vi "Update UI row elements.vi"(8 "result":string="Pass", 9 "measured value":string="Started", 11 "input cluster":T1={"User name"="", "user account"="", "UI"=[], "DI"=[], "Barcode"="", "MCListbox Ref_in"=refnum, "sequence step #"=0, "Result?"=FALSE, "Report Path"=path "", "Test Sequence"=enum."Ensure all the connections are OK", "skip Test  "=[FALSE, FALSE, FALSE, FALSE, FALSE, FALSE, FALSE, FALSE, FALSE, FALSE, FALSE, FALSE, FALSE, FALSE, FALSE, FALSE, FALSE, FALSE, FALSE, FALSE, FALSE, FALSE, FALSE, FALSE, FALSE, FALSE, FALSE, FALSE, FALSE, FALSE, FALSE, FALSE]} {"DI"."Upper limit" format="%#_7f"; "DI"."Lower limit" format="%#_7f"}) -> (1 "Test status item names":string[][](array[string]), 3 "output cluster":T1={"User name"="", "user account"="", "UI"=[], "DI"=[], "Barcode"="", "MCListbox Ref_in"=refnum, "sequence step #"=0, "Result?"=FALSE, "Report Path"=path "", "Test Sequence"=enum."Ensure all the connections are OK", "skip Test  "=[FALSE, FALSE, FALSE, FALSE, FALSE, FALSE, FALSE, FALSE, FALSE, FALSE, FALSE, FALSE, FALSE, FALSE, FALSE, FALSE, FALSE, FALSE, FALSE, FALSE, FALSE, FALSE, FALSE, FALSE, FALSE, FALSE, FALSE, FALSE, FALSE, FALSE, FALSE, FALSE]} {"DI"."Upper limit" format="%#_7f"; "DI"."Lower limit" format="%#_7f"})   [LabVIEW 2021]
uses:
  5.ACTIVITIES/1.LabVIEW_State_Machine_Template/LabVIEW_State_Machine_Template/LabVIEW_State_Machine_Template/Project_Template/Queue Test updator/Controls/initialise cluster.ctl
  5.ACTIVITIES/1.LabVIEW_State_Machine_Template/LabVIEW_State_Machine_Template/LabVIEW_State_Machine_Template/Project_Template/Queue Test updator/Controls/test step description.ctl
  5.ACTIVITIES/1.LabVIEW_State_Machine_Template/LabVIEW_State_Machine_Template/LabVIEW_State_Machine_Template/Project_Template/Queue Test updator/Controls/comparison selection.ctl
  controls/Main test sequence.ctl
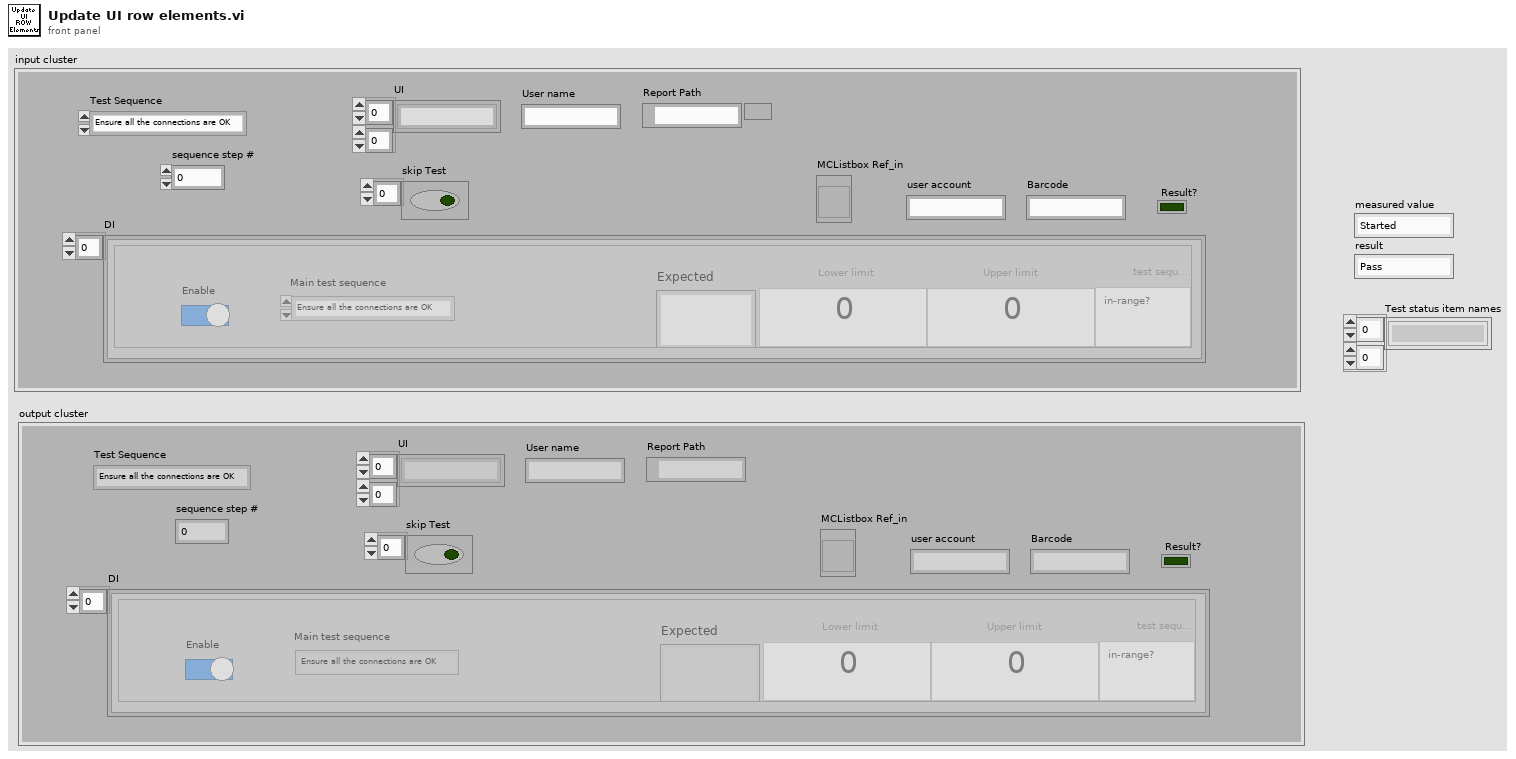
[diagram p1: front panel]
types:
  T1 = typedef "initialise cluster.ctl" = cluster{"User name":string, "user account":string, "UI":string[][], "DI":T2[], "Barcode":string, "MCListbox Ref_in":refnum<vi>, "sequence step #":u32, "Result?":bool, "Report Path":path, "Test Sequence":T4, "skip Test  ":bool[]}
  T2 = typedef "test step description.ctl" = cluster{"Lower limit":dbl, "Upper limit":dbl, "Comparison":T3, "Expected":string, "Enable":bool, "Main test sequence":T4}
  T3 = typedef "comparison selection.ctl" = enum16{"None", "in-range?", "less than?", "greater than?", "equal to?", "not equal to?", "less or equal to?", "greater or equal to?"}
  T4 = typedef "Main test sequence.ctl" = enum16{"Initialization", "Ensure all the connections are OK", "Turn ON 230V AC Input", "Load the Firmware", "Unlock_Opensesame & Stop console Logs", "Earth Detection", "Read Firmware", "Read & Write PCB Serial No", "Emergancy Switch Check", "Update WIFI credentials ", "Reboot", "Unlock Opensesame & Stop_console Logs", "WIFI State", "WIFI SSID", "Board revision", "ADC NTC Temp", "ADC_TYPE2_RCD_CURRENT", "5V Output Voltage", "3.3V Output Voltage", "D+M Sense", "Output Weld Sense", "FW Power Reset", "Unlock Opensesame & Stop console_Logs", "Reset switch Check", "Exit"}
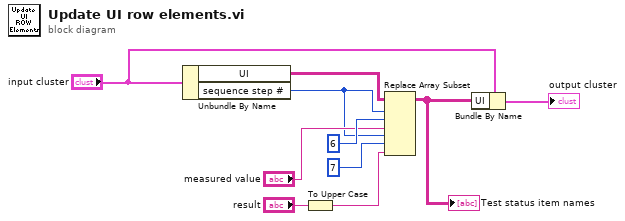
[diagram p0: block diagram]
diagram:
  n1 = Unbundle By Name("input cluster") -> ("UI"=w9:string[][], "sequence step #"=w1:u32)
  n2 = To Upper Case(1:"result") -> (0:w2:string)
  n3 = Replace Array Subset(array=w9, new element #1="measured value", index (row) #1=w1, index (col) #1=6 ("disabled index (col)"), new element #2=w2, index (row) #2=w1, index (col) #2=7 ("disabled index (col)")) -> (w4:string[][])
  "Test status item names" <- w4
  n4 = Bundle By Name(cluster="input cluster", "UI"=w4) -> (→"output cluster":T1)
